vi "Cmd_Read.vi"(6 "Refnum in":refnum<k21>, 8 "error in (no error)":errorcluster) -> (0 "error out":errorcluster, 1 "timed out?":bool, 2 "data out":T1, 4 "Refnum out":refnum<k21>)   [LabVIEW 2025]
uses:
  Command.ctl
  vi/thresholds.ctl
  RT_Cmd.ctl
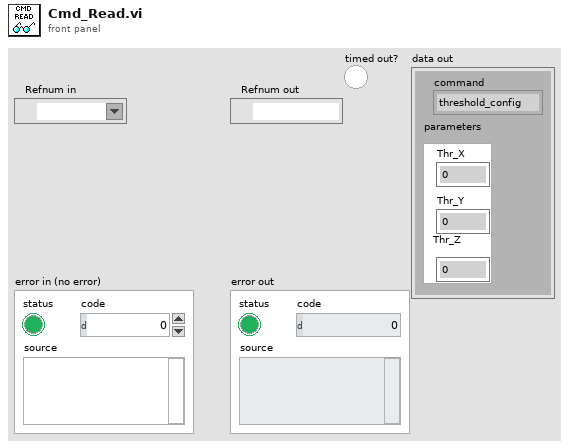
[diagram p1: front panel]
types:
  T1 = typedef "RT_Cmd.ctl" = cluster{"command":T2, "parameters":T3}
  T2 = typedef "Command.ctl" = enum16{"threshold_config", "manual_trigger", "stop"}
  T3 = typedef "thresholds.ctl" = cluster{"Thr_X":i16, "Thr_Y":i16, "Thr_Z":i16}
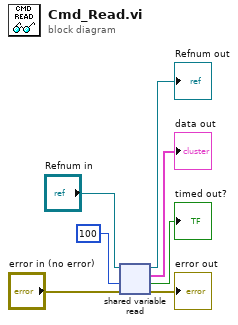
[diagram p0: block diagram]
diagram:
  n1 = shared-variable-read("Refnum in", "error in (no error)", 100 ("timeout ms (-1)")) -> (→"Refnum out":refnum<k21>, →"error out":errorcluster, →"timed out?":bool, →"data out":T1)
